vi "test-find-path.vi"() -> ()   [LabVIEW 2019]
uses:
  <vilib>/Rock Robotics/WPI/ThirdParty/JAS_Junk/TrajLib/TypeDef/TRANSLATION2D.ctl
  <vilib>/Rock Robotics/WPI/ThirdParty/MJansen/PathPlanner/TypeDef/PathPlannerGoalEndState.ctl
  <vilib>/Rock Robotics/WPI/ThirdParty/JAS_Junk/TrajLib/TypeDef/ROTATION2D.ctl
  <vilib>/Rock Robotics/WPI/ThirdParty/MJansen/PathPlanner/TypeDef/PathPlannerPath.ctl
  <vilib>/Rock Robotics/WPI/ThirdParty/MJansen/PathPlanner/TypeDef/PathPlannerRotationTarget.ctl
  <vilib>/Rock Robotics/WPI/ThirdParty/MJansen/PathPlanner/TypeDef/PathPlannerConstraintsZone.ctl
  <vilib>/Rock Robotics/WPI/ThirdParty/MJansen/PathPlanner/TypeDef/PathPlannerPathConstraints.ctl
  <vilib>/Rock Robotics/WPI/ThirdParty/MJansen/PathPlanner/TypeDef/PathPlannerEventMarker.ctl
  <vilib>/Rock Robotics/WPI/ThirdParty/MJansen/PathPlanner/TypeDef/PathPlannerCommandUtil.ctl
  <vilib>/Rock Robotics/WPI/ThirdParty/MJansen/PathPlanner/ENum/PathPlanner_CommandUtilType_ENUM.ctl
  <vilib>/Rock Robotics/WPI/ThirdParty/MJansen/PathPlanner/TypeDef/PathPlannerPathPoint.ctl
  <vilib>/Rock Robotics/WPI/ThirdParty/MJansen/PathPlanner/TypeDef/PathPlannerWaypoint.ctl
  <vilib>/Rock Robotics/WPI/ThirdParty/MJansen/PathPlanner/TypeDef/PathPlannerPointTowardsZone.ctl
  <vilib>/Rock Robotics/WPI/ThirdParty/MJansen/PathPlanner/TypeDef/PathPlannerIdealStartingState.ctl
  <vilib>/Rock Robotics/WPI/ThirdParty/JAS_Junk/TrajLib/TypeDef/CHASSIS_SPEEDS.ctl
  <vilib>/Rock Robotics/WPI/ThirdParty/MJansen/PathPlanner/VI/PathPlanner_GridPosition_Get.vi
  <vilib>/Rock Robotics/WPI/ThirdParty/JAS_Junk/TrajLib/Translation2d_Create.vi
  <vilib>/Rock Robotics/WPI/ThirdParty/MJansen/PathPlanner/VI/PathPlanner_PathFinder_Globals.vi
  <vilib>/robotics/Navigation/shared/WorldMap/OccupancyGridWorldMap/NI_Robotics_OccupancyGridWorldMap.lvclass
  <vilib>/robotics/Navigation/shared/MapNode/AbstractDstarNode/NI_Robotics_AbstractDstarNode.lvclass
  <vilib>/Rock Robotics/WPI/ThirdParty/MJansen/PathPlanner/PathPlanner24.lvlib
  <vilib>/Rock Robotics/WPI/ThirdParty/JAS_Junk/TrajLib/Trajectory_Library.lvlib
panel:
  out "Extract Simplified Path Size":i32
  out "Do Reset Err Count":i64
  out "Do Minor Err Count":i64
  out "Do Major Err Count":i64
  out "Extract Path Size":i32
  out "Field":cluster{dbl[], dbl[]}[](graph)
  out "Error_No_Path":bool
  out "New Path Available":bool
  out "Loop Count":i32
  out "TerminateWorker":bool
  out "Do Work Count":i64
  out "Do Reset Count":i64
  out "Do Minor Count":i64
  out "Do Major Count":i64
  out "PathPlannerPath":T1={"Reversed"=FALSE, "RotationTargets"=[], "ConstraintZones"=[], "EventMarkers"=[], "GlobalConstraints"={"MaxVelocityMps;"=0.0, "MaxAccelerationMpsSq;"=0.0, "MaxAngularVelRadPsEc;"=0.0, "MaxAngularAccRadPSecSq"=0.0, "Exists"=FALSE, "Unlimited"=FALSE, "NominalVoltageVolts"=1.0}, "GoalEndState"={"VelocityMPS"=0.0, "Rotation"={"VALUE"=0.0, "COS"=1.0, "SIN"=0.0}}, "AllPoints"=[], "Name"="", "Waypoints"=[], "PointTowardsZones"=[], "IdealStartingState"={"VelocityMPS"=0.0, "Rotation"={"VALUE"=0.0, "COS"=1.0, "SIN"=0.0}}, "IsChoreoPath"=FALSE, "PreventFlipping"=FALSE} {"IdealStartingState"."Rotation"."SIN" format="%13.4f"; "IdealStartingState"."Rotation"."COS" format="%13.4f"; "IdealStartingState"."Rotation"."VALUE" format="%13.4f"; "PointTowardsZones"."TargetPosition"."Y" format="%14.3f"; "PointTowardsZones"."TargetPosition"."X" format="%14.3f"; "PointTowardsZones"."RotationOffset"."SIN" format="%13.4f"; "PointTowardsZones"."RotationOffset"."COS" format="%13.4f"; "PointTowardsZones"."RotationOffset"."VALUE" format="%13.4f"; "Waypoints"."nextControl"."Y" format="%14.3f"; "Waypoints"."nextControl"."X" format="%14.3f"; "Waypoints"."anchor"."Y" format="%14.3f"; "Waypoints"."anchor"."X" format="%14.3f"; "Waypoints"."prevControl"."Y" format="%14.3f"; "Waypoints"."prevControl"."X" format="%14.3f"; "AllPoints"."RotationTarget"."rotation"."SIN" format="%13.4f"; "AllPoints"."RotationTarget"."rotation"."COS" format="%13.4f"; "AllPoints"."RotationTarget"."rotation"."VALUE" format="%13.4f"; "AllPoints"."Position"."Y" format="%14.3f"; "AllPoints"."Position"."X" format="%14.3f"; "GoalEndState"."Rotation"."SIN" format="%13.4f"; "GoalEndState"."Rotation"."COS" format="%13.4f"; "GoalEndState"."Rotation"."VALUE" format="%13.4f"; "RotationTargets"."rotation"."SIN" format="%13.4f"; "RotationTargets"."rotation"."COS" format="%13.4f"; "RotationTargets"."rotation"."VALUE" format="%13.4f"}
  in  "GoalEndState":T9={"VelocityMPS"=0.0, "Rotation"={"VALUE"=0.0, "COS"=1.0, "SIN"=0.0}} {"Rotation"."SIN" format="%13.4f"; "Rotation"."COS" format="%13.4f"; "Rotation"."VALUE" format="%13.4f"}
  in  "Goal Position":T11={"X"=14.0, "Y"=7.0} {"Y" step=0.25 format="%14.3f"; "X" step=0.25 format="%14.3f"}
  in  "StartPosition":T11={"X"=1.5, "Y"=1.5} {"Y" step=0.25 format="%14.3f"; "X" step=0.25 format="%14.3f"}
  out "NewPathAvailLastCheck":i32
  out "NewPathAvailCount":i32
  out "BackGroundInitialized":bool
  out "Main Program Name":string
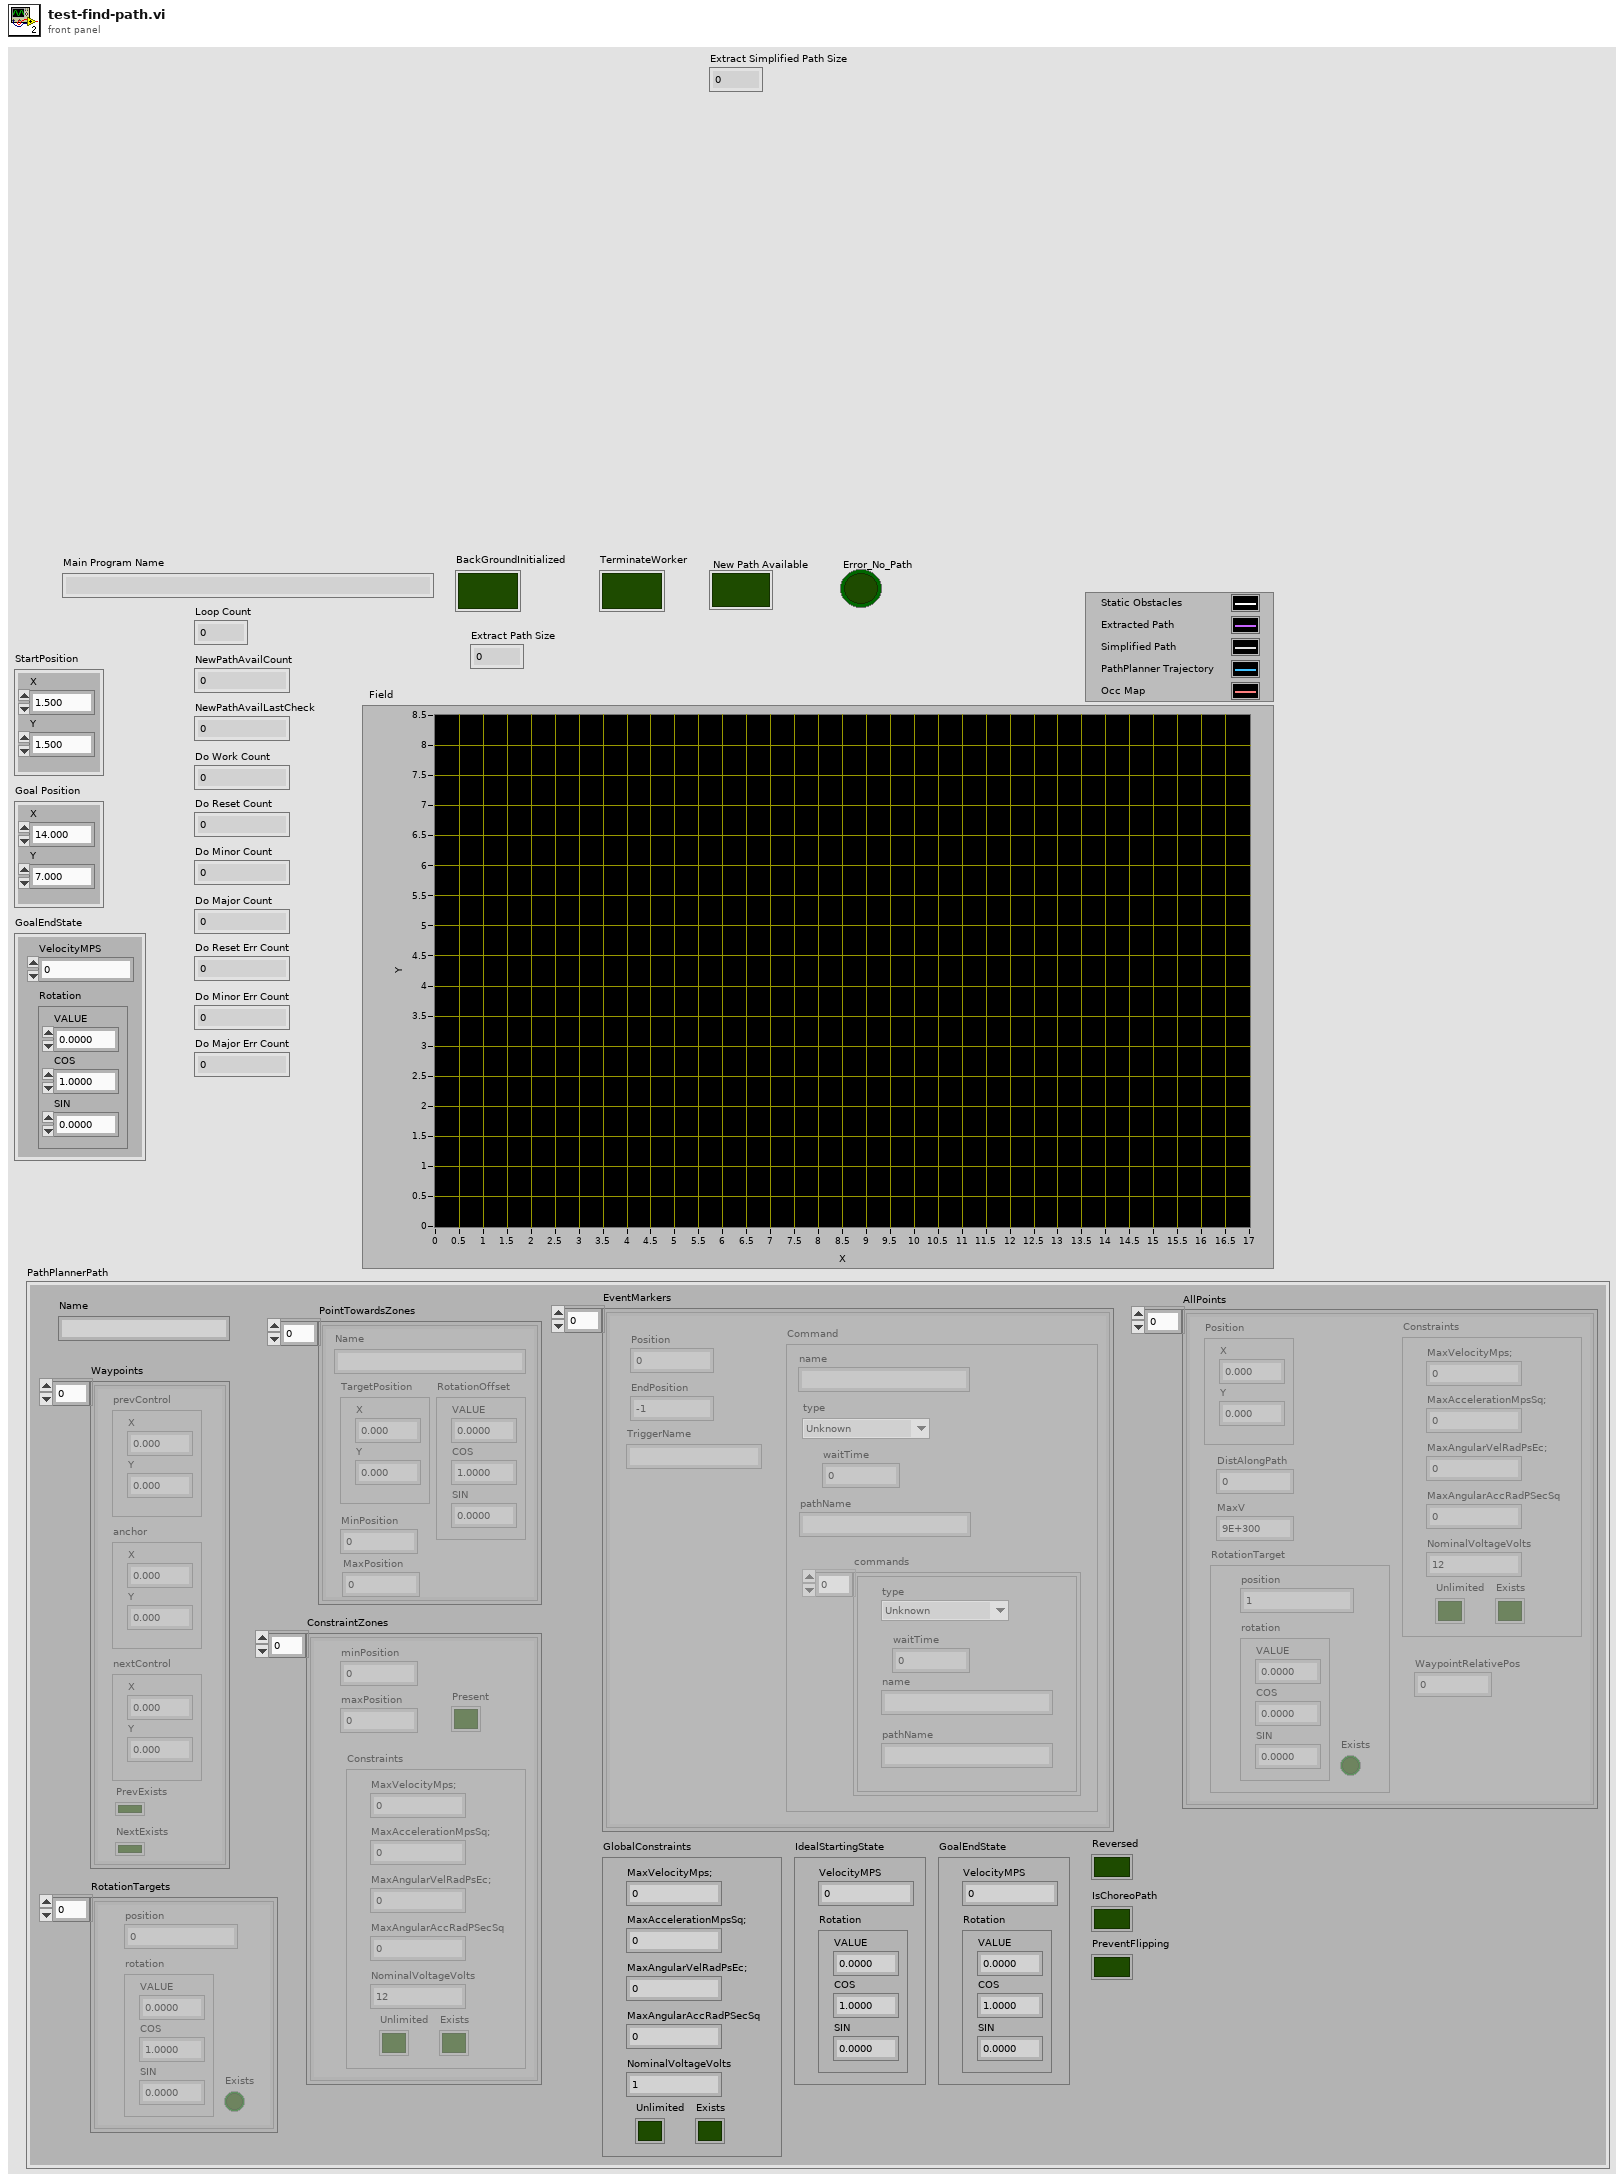
[diagram p1: front panel]
types:
  T1 = typedef "PathPlanner24.lvlib/PathPlannerPath.ctl" = cluster{"Reversed":bool, "RotationTargets":T2[], "ConstraintZones":T4[], "EventMarkers":T6[], "GlobalConstraints":T5, "GoalEndState":T9, "AllPoints":T10[], "Name":string, "Waypoints":T12[], "PointTowardsZones":T13[], "IdealStartingState":T14, "IsChoreoPath":bool, "PreventFlipping":bool}
  T2 = typedef "PathPlanner24.lvlib/PathPlannerRotationTarget.ctl" = cluster{"position":dbl, "rotation":T3, "Exists":bool}
  T3 = typedef "Trajectory_Library.lvlib/ROTATION2D.ctl" = cluster{"VALUE":dbl, "COS":dbl, "SIN":dbl}
  T4 = typedef "PathPlanner24.lvlib/PathPlannerConstraintsZone.ctl" = cluster{"minPosition":dbl, "maxPosition":dbl, "Constraints":T5, "Present":bool}
  T5 = typedef "PathPlanner24.lvlib/PathPlannerPathConstraints.ctl" = cluster{"MaxVelocityMps;":dbl, "MaxAccelerationMpsSq;":dbl, "MaxAngularVelRadPsEc;":dbl, "MaxAngularAccRadPSecSq":dbl, "Exists":bool, "Unlimited":bool, "NominalVoltageVolts":dbl}
  T6 = typedef "PathPlanner24.lvlib/PathPlannerEventMarker.ctl" = cluster{"Position":dbl, "Command":T7, "TriggerName":string, "EndPosition":dbl}
  T7 = typedef "PathPlanner24.lvlib/PathPlannerCommandUtil.ctl" = cluster{"waitTime":dbl, "name":string, "pathName":string, "commands":cluster{"type":T8, "waitTime":dbl, "name":string, "pathName":string}[], "type":T8}
  T8 = typedef "PathPlanner24.lvlib/PathPlanner_CommandUtilType_ENUM.ctl" = enum16{"Unknown", "Wait", "Named", "Path", "Sequential", "Parallel", "Race", "Deadline"}
  T9 = typedef "PathPlanner24.lvlib/PathPlannerGoalEndState.ctl" = cluster{"VelocityMPS":dbl, "Rotation":T3}
  T10 = typedef "PathPlanner24.lvlib/PathPlannerPathPoint.ctl" = cluster{"Position":T11, "DistAlongPath":dbl, "MaxV":dbl, "Constraints":T5, "RotationTarget":T2, "WaypointRelativePos":dbl}
  T11 = typedef "Trajectory_Library.lvlib/TRANSLATION2D.ctl" = cluster{"X":dbl, "Y":dbl}
  T12 = typedef "PathPlanner24.lvlib/PathPlannerWaypoint.ctl" = cluster{"prevControl":T11, "anchor":T11, "nextControl":T11, "PrevExists":bool, "NextExists":bool}
  T13 = typedef "PathPlanner24.lvlib/PathPlannerPointTowardsZone.ctl" = cluster{"RotationOffset":T3, "Name":string, "TargetPosition":T11, "MinPosition":dbl, "MaxPosition":dbl}
  T14 = typedef "PathPlanner24.lvlib/PathPlannerIdealStartingState.ctl" = cluster{"VelocityMPS":dbl, "Rotation":T3}
  T15 = typedef "Trajectory_Library.lvlib/CHASSIS_SPEEDS.ctl" = cluster{"vX":dbl, "vY":dbl, "vOmega":dbl}
  T16 = cluster{"DoResetErrCount":i64, "DoResetCount":i64, "DoMinorErrCount":i64, "DoMinorCount":i64, "DoMajorErrCount":i64, "DoMajorCount":i64, "DoWorkLoopCount":i64, "BackGroundInitialized":bool, "TerminateWorker":bool}
  T17 = typedef "PathPlanner24.lvlib/PathPlannerFinderGridPosition.ctl" = cluster{"X":i32, "Y":i32}
  T18 = cluster{"ExtractedPath":T17[], "ExtractedPathSimplified":T17[], "ExtractedFieldPosPath":T11[], "CurrentPath":T11[], "Obstacles":set{T17}, "StaticOccupancyGrid":refnum<data-value>, "path references":refnum<data-value>[], "Main Program Name":string}
  T19 = typedef "PathPlanner24.lvlib/PathPlannerTrajectory.ctl" = cluster{"States":T20[]}
  T20 = typedef "PathPlanner24.lvlib/PathPlannerTrajectoryState.ctl" = cluster{"TimeSeconds":dbl, "VelocityMPS":dbl, "AccerationMpsSq":dbl, "HeadingAngularVelRadPerSec":dbl, "PositionMeters":T11, "Heading":T3, "TargetHolonomicRotation":T3, "CurvatureRadPerMeter":dbl, "PathPlannerConstraints":T5, "DeltaPos":dbl}
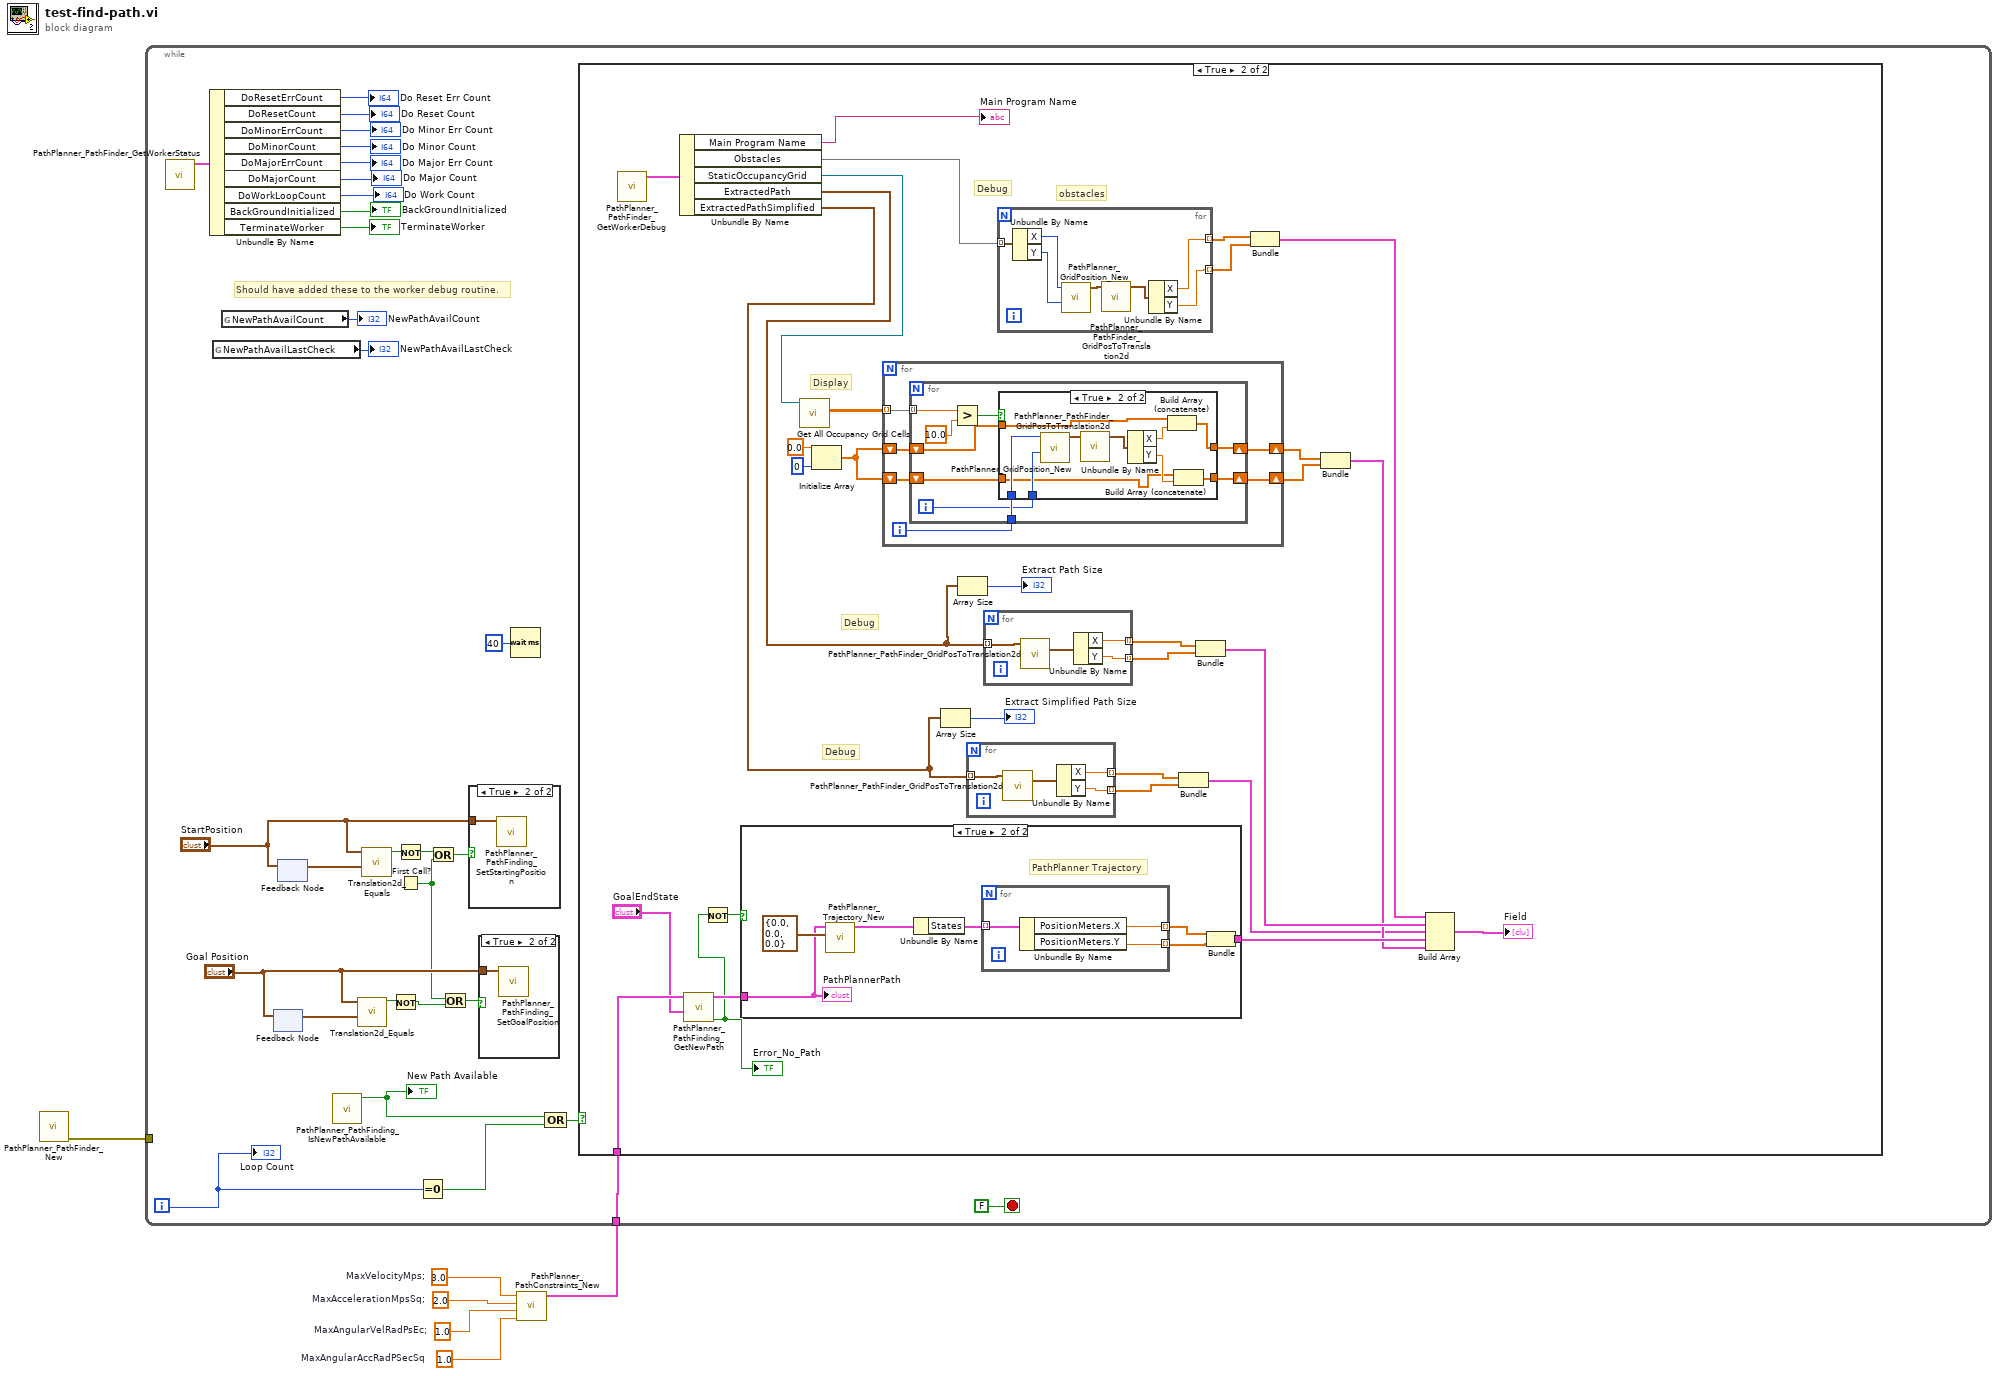
[diagram p0: block diagram]
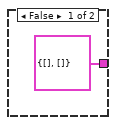
[diagram p3: hidden frame]
diagram:
  w2 = 3.0  # MaxVelocityMps;
  w3 = 2.0  # MaxAccelerationMpsSq;
  w4 = 1.0  # MaxAngularVelRadPsEc;
  w5 = 1.0  # MaxAngularAccRadPSecSq
  n1 = call <vilib>:"PathPlanner_PathFinder_New.vi"() -> ("error out"=w1:errorcluster)  [unwired: 11 in]
  n2 = call <vilib>:"PathPlanner_PathConstraints_New.vi"("MaxAngularAccRadPSecSq"=w5, "MaxAngularVelRadPsEc;"=w4, "MaxAccelerationMpsSq;"=w3, "MaxVelocityMps;"=w2) -> ("PathPlannerConstraints"=w6:T5)  [unwired: 7 in]
  n3 = while {
    tunnel: w6 -> [w29]
    tunnel: w1 -> [_]
    i -> [w31]
    stop <- FALSE stop-if-true
    # "Should have added these to the worker debug routine."
    n4 = call <vilib>:"PathPlanner_PathFinder_GetWorkerStatus.vi"() -> ("PathFindingWorkerStatus"=w16:T16)  [unwired: 11 in]
    n5 = Unbundle By Name(w16) -> ("DoResetErrCount"=→"Do Reset Err Count":i64, "DoResetCount"=→"Do Reset Count":i64, "DoMinorErrCount"=→"Do Minor Err Count":i64, "DoMinorCount"=→"Do Minor Count":i64, "DoMajorErrCount"=→"Do Major Err Count":i64, "DoMajorCount"=→"Do Major Count":i64, "DoWorkLoopCount"=→"Do Work Count":i64, "BackGroundInitialized"=→"BackGroundInitialized":bool, "TerminateWorker"=→"TerminateWorker":bool)
    n6 = global read "PathPlanner_PathFinder_Globals.vi" "NewPathAvailLastCheck"() -> (→"NewPathAvailLastCheck":i32)
    n7 = global read "PathPlanner_PathFinder_Globals.vi" "NewPathAvailCount"() -> (→"NewPathAvailCount":i32)
    n8 = feedback #1() -> (w33:T11)  [unwired: 1 in]
    n9 = feedback-in #1("Goal Position") -> ()
    n10 = feedback-in #2("StartPosition") -> ()
    n11 = feedback #2() -> (w35:T11)  [unwired: 1 in]
    n12 = call <vilib>:"PathPlanner_PathFinding_IsNewPathAvailable.vi"() -> ("New Path Available"=w26:bool)  [unwired: 10 in, 1 out]
    "New Path Available" <- w26
    n13 = call <vilib>:"Translation2d_Equals.vi"("other Translation"=w33, "In Translation"="Goal Position") -> ("Equals"=w32:bool)  [unwired: 9 in]
    n14 = call <vilib>:"Translation2d_Equals.vi"("other Translation"=w35, "In Translation"="StartPosition") -> ("Equals"=w34:bool)  [unwired: 9 in]
    n15 = Not(x=w32) -> (.not. x?=w21:bool)
    n16 = Not(x=w34) -> (.not. x?=w19:bool)
    n17 = First Call?() -> (First Call?: T/F=w20:bool)
    n18 = Equal To 0?(x=w31) -> (x = 0?=w28:bool)
    n19 = Or(x=w19, y=w20) -> (x .or. y?=w23:bool)
    n20 = Or(x=w20, y=w21) -> (x .or. y?=w22:bool)
    n21 = case shown="True" w23 {
      tunnel: "StartPosition" -> [_ w122]
      frame False {
      }
      frame True {
        n22 = call <vilib>:"PathPlanner_PathFinding_SetStartingPosition.vi"("StartPosition"=w122) -> ()  [unwired: 10 in, 1 out]
      }
    }
    n23 = case shown="True" w22 {
      tunnel: "Goal Position" -> [_ w121]
      frame False {
      }
      frame True {
        n24 = call <vilib>:"PathPlanner_PathFinding_SetGoalPosition.vi"("GoalPosition"=w121) -> ()  [unwired: 10 in, 1 out]
      }
    }
    n25 = Wait (ms)(milliseconds to wait=u32 40) -> ()  [unwired: 1 out]
    n26 = Compound Arithmetic op=OR(w26, w28) -> (w30:bool)
    n27 = case shown="True" w30 {
      tunnel: w29 -> [_ w62]
      frame False {
      }
      frame True {
        # "Debug"
        # "Display"
        # "Debug"
        # "Debug"
        # "obstacles"
        n28 = call <vilib>:"PathPlanner_PathFinder_GetWorkerDebug.vi"() -> ("PathFinderWorkerDebug"=w44:T18)  [unwired: 11 in]
        n29 = Unbundle By Name(w44) -> ("Main Program Name"=→"Main Program Name":string, "Obstacles"=w42:set{T17}, "StaticOccupancyGrid"=w41:refnum<data-value>, "ExtractedPath"=w40:T17[], "ExtractedPathSimplified"=w39:T17[])
        n30 = call <vilib>:"PathPlanner_PathFinding_GetNewPath.vi"("GoalEndState"="GoalEndState", "PathPlannerPathConstraints"=w62) -> ("Error_No_Path"=w37:bool, "PathPlannerPath"=w60:T1)  [unwired: 8 in]
        "Error_No_Path" <- w37
        n31 = Not(x=w37) -> (.not. x?=w38:bool)
        n32 = case shown="True" w38 {
          tunnel: w60 -> [_ w73]
          tunnel: [cluster{dbl[], dbl[]} {[], []} w69] -> w57
          frame False {
          }
          frame True {
            # "PathPlanner Trajectory"
            n33 = call <vilib>:"PathPlanner_Trajectory_New.vi"("StartingSpeeds"=T15 {"vX"=0.0, "vY"=0.0, "vOmega"=0.0}, "Path"=w73) -> ("PathPlannerTrajectory"=w74:T19)  [unwired: 8 in, 1 out]
            n34 = Unbundle By Name(w74) -> ("States"=w72:T20[])
            n35 = for {
              tunnel: [w77] -> w71 mode=indexing
              tunnel: [w78] -> w70 mode=indexing
              tunnel: w72 -> [w76] mode=indexing
              n36 = Unbundle By Name(w76) -> ("PositionMeters.X"=w77:dbl, "PositionMeters.Y"=w78:dbl)
            }
            n37 = Bundle(w71, w70) -> (w69:cluster{dbl[], dbl[]})  [unwired: 1 in]
            "PathPlannerPath" <- w73
          }
        }
        n38 = call <vilib>:"Get All Occupancy Grid Cells.vi"("map reference in"=w41) -> ("occupancy grid"=w48:dbl[][])  [unwired: 8 in, 2 out]
        n39 = Initialize Array(0.0 ("element"), 0 ("dimension size")) -> (w45:dbl[])
        n40 = for {
          tunnel: w48 -> [w88] mode=indexing
          shift-right: [w84] -> w55
          shift-left: w45 -> [w87]
          shift-right: [w83] -> w54
          shift-left: w45 -> [w86]
          i -> [w85]
          n41 = for {
            tunnel: w88 -> [w97] mode=indexing
            shift-right: [w91] -> w84
            shift-left: w87 -> [w92]
            shift-right: [w89] -> w83
            shift-left: w86 -> [w90]
            tunnel: w85 -> [w94]
            i -> [w93]
            n42 = Greater?(x=w97, y=10.0) -> (0:w95:bool)
            n43 = case shown="True" w95 {
              tunnel: w94 -> [_ w108]
              tunnel: w93 -> [_ w104]
              tunnel: w92 -> [w99 w103]
              tunnel: [w99 w102] -> w91
              tunnel: w90 -> [w98 w101]
              tunnel: [w98 w100] -> w89
              frame False {
              }
              frame True {
                n44 = call <vilib>:"PathPlanner_GridPosition_New.vi"("Int Y"=w104, "Int X"=w108) -> ("GridPosition"=w109:T17)  [unwired: 9 in]
                n45 = call <vilib>:"PathPlanner_PathFinder_GridPosToTranslation2d.vi"("GridPosition"=w109) -> ("RealGridPos"=w107:T11)  [unwired: 10 in]
                n46 = Unbundle By Name(w107) -> ("X"=w106:dbl, "Y"=w105:dbl)
                n47 = Build Array (concatenate)(w103, w106) -> (w102:dbl[])
                n48 = Build Array (concatenate)(w101, w105) -> (w100:dbl[])
              }
            }
          }
        }
        n49 = Array Size(array=w39) -> (size(s)=→"Extract Simplified Path Size":i32)
        n50 = Array Size(array=w40) -> (size(s)=→"Extract Path Size":i32)
        n51 = for {
          tunnel: [w80] -> w52 mode=indexing
          tunnel: [w82] -> w51 mode=indexing
          tunnel: w39 -> [w79] mode=indexing
          n52 = call <vilib>:"PathPlanner_PathFinder_GridPosToTranslation2d.vi"("GridPosition"=w79) -> ("RealGridPos"=w81:T11)  [unwired: 10 in]
          n53 = Unbundle By Name(w81) -> ("X"=w80:dbl, "Y"=w82:dbl)
        }
        n54 = for {
          tunnel: [w111] -> w59 mode=indexing
          tunnel: [w113] -> w58 mode=indexing
          tunnel: w40 -> [w110] mode=indexing
          n55 = call <vilib>:"PathPlanner_PathFinder_GridPosToTranslation2d.vi"("GridPosition"=w110) -> ("RealGridPos"=w112:T11)  [unwired: 10 in]
          n56 = Unbundle By Name(w112) -> ("X"=w111:dbl, "Y"=w113:dbl)
        }
        n57 = for {
          tunnel: w42 -> [w120] mode=indexing
          tunnel: [w115] -> w66 mode=indexing
          tunnel: [w114] -> w67 mode=indexing
          n58 = Unbundle By Name(w120) -> ("X"=w117:i32, "Y"=w116:i32)
          n59 = call <vilib>:"PathPlanner_GridPosition_New.vi"("Int Y"=w116, "Int X"=w117) -> ("GridPosition"=w119:T17)  [unwired: 9 in]
          n60 = call <vilib>:"PathPlanner_PathFinder_GridPosToTranslation2d.vi"("GridPosition"=w119) -> ("RealGridPos"=w118:T11)  [unwired: 10 in]
          n61 = Unbundle By Name(w118) -> ("X"=w115:dbl, "Y"=w114:dbl)
        }
        n62 = Bundle(w52, w51) -> (w49:cluster{dbl[], dbl[]})  [unwired: 1 in]
        n63 = Bundle(w59, w58) -> (w63:cluster{dbl[], dbl[]})  [unwired: 1 in]
        n64 = Bundle(w66, w67) -> (w64:cluster{dbl[], dbl[]})  [unwired: 1 in]
        n65 = Bundle(w55, w54) -> (w56:cluster{dbl[], dbl[]})  [unwired: 1 in]
        n66 = Build Array(w64, w63, w49, w57, w56) -> (→"Field":cluster{dbl[], dbl[]}[])
      }
    }
    "Loop Count" <- w31
  }
